vi "csb bit timing.vi"(0 "nominal_bitrate":u32, 1 "timing":u16[](array[numeric])=[0, 0, 0, 0, 0, 0, 0, 0], 5 "nominal_sp":dbl, 7 "data_bitrate":u32, 9 "data_sp":dbl, 11 "error in (no error)":errorcluster) -> (3 "timing out":u16[](array[numeric]), 4 "nominal_sp_out":dbl, 6 "data_sp_out":dbl, 8 "function return":i32, 15 "error out":errorcluster)   [LabVIEW 2021, in "CANsub_Codec.lvlib"]
doc: "int32_t csb_bit_timing(uint32_t nominal_bitrate, double nominal_sp,\n uint32_t data_bitrate, double data_sp,\n uint16_t *timing, double *nominal_sp_out, double *data_sp_out);"
uses:
  CANsub_Codec.lvlib
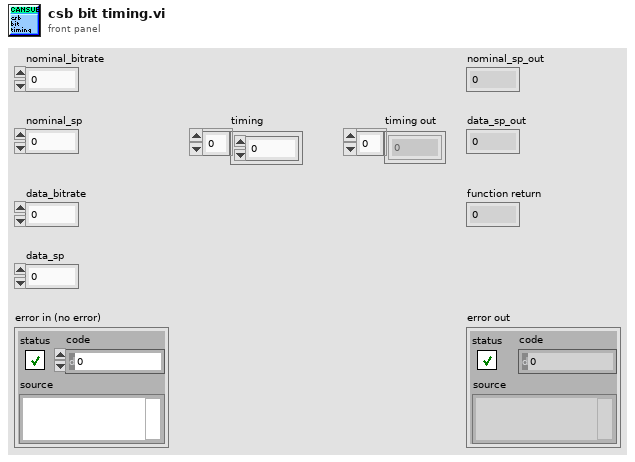
[diagram p1: front panel]
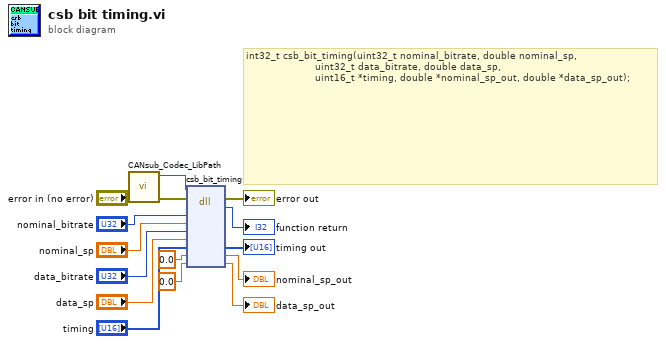
[diagram p0: block diagram]
diagram:
  # "int32_t csb_bit_timing(uint32_t nominal_bitrate, double nominal_sp,\n                       uint32_t data_bitrate, double data_sp,\n                       uint16_t *timing, double *nominal_sp_out, double *data_sp_out);"
  n1 = call "CANsub_Codec_LibPath.vi"() -> ("Path"=w1:path)  [unwired: 11 in]
  n2 = dll-call lib="libcansub_codec.*" fn="csb_bit_timing"(path in=w1, error in="error in (no error)", "nominal_bitrate"="nominal_bitrate", "nominal_sp"="nominal_sp", "data_bitrate"="data_bitrate", "data_sp"="data_sp", "timing"="timing", "nominal_sp_out"=0.0, "data_sp_out"=0.0) -> (error out=→"error out":errorcluster, "return type"=→"function return":i32, "timing"=→"timing out":u16[], "nominal_sp_out"=→"nominal_sp_out":dbl, "data_sp_out"=→"data_sp_out":dbl)  [unwired: 5 in, 1 out]
